vi "FX_Test.vi"() -> ()   [LabVIEW 2018]
doc: "Use this template to build a VI to use as a subVI."
panel:
  out "error out":errorcluster
  out "Words":u16[](array[numeric])
  in  "Read Count":u16
  in  "Read Device":string
  in  "Word Value":u16
  in  "Word Device":string
  in  "Port":u16
  in  "Host":string
  # "說明：單獨測通訊用，固定走 TCP，只給模擬器。"
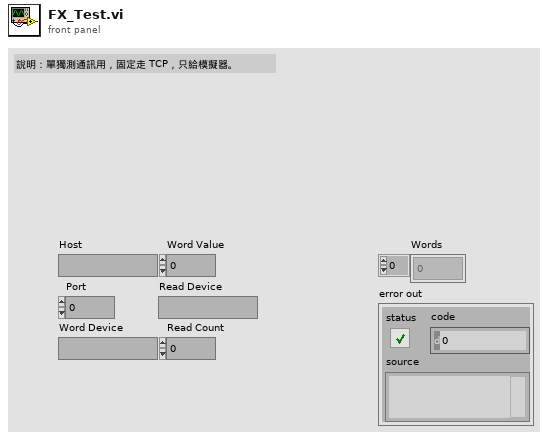
[diagram p1: front panel]
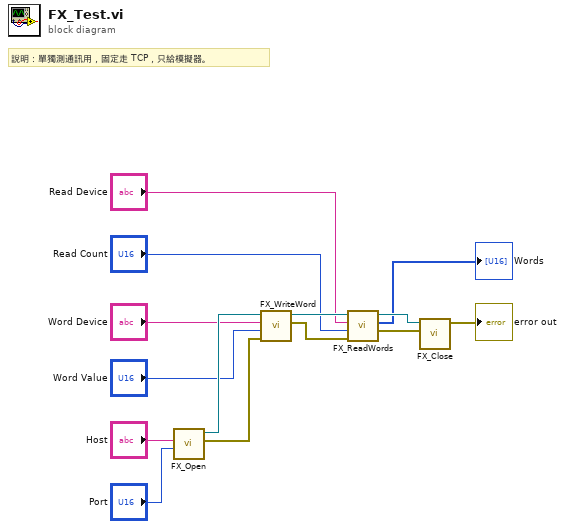
[diagram p0: block diagram]
diagram:
  # "說明：單獨測通訊用，固定走 TCP，只給模擬器。"
  n1 = call "FX_Open.vi"("Port"="Port", "Host"="Host") -> ("error out"=w13:errorcluster, "PLC Conn"=w14:refnum<visa-resource-name>)  [unwired: 8 in]
  n2 = call "FX_WriteWord.vi"("error in (no error)"=w13, "Value"="Word Value", "Device"="Word Device", "PLC Conn"=w14) -> ("error out"=w11:errorcluster, "PLC Conn out"=w12:refnum<visa-resource-name>)  [unwired: 6 in]
  n3 = call "FX_ReadWords.vi"("error in (no error)"=w11, "Count"="Read Count", "Device"="Read Device", "PLC Conn"=w12) -> ("error out"=w9:errorcluster, "Words"=→"Words":u16[], "PLC Conn out"=w10:refnum<visa-resource-name>)  [unwired: 5 in]
  n4 = call "FX_Close.vi"("error in (no error)"=w9, "PLC Conn"=w10) -> ("error out"=→"error out":errorcluster)  [unwired: 9 in]
